vi "prepare_keyboard_notes.vi"(7 "Anticlockwise rotations [0-3] (0)":i32, 8 "error in (no error)":errorcluster, 9 "Note Length (-1)":dbl=-1.0, 10 "Total Length (1200)":dbl=1200.0, 11 "midi-ui in":refnum<class "midi-ui.lvclass">) -> (0 "error out":errorcluster, 3 "midi-ui out":refnum<class "midi-ui.lvclass">)   [LabVIEW 2020, in "midi-ui.lvclass"]
uses:
  midi-ui.lvclass
  midi-ui.lvclass/midi-ui.ctl
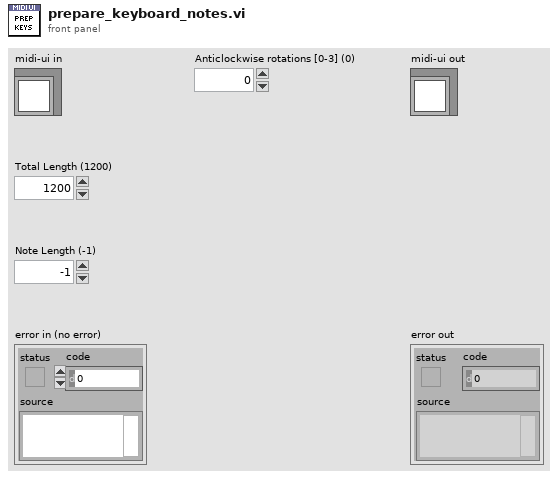
[diagram p1: front panel]
types:
  T1 = typedef "midi-ui.lvclass/privatedata.ctl" = cluster{"White Key Length":dbl, "White Key Width":dbl, "Black Key Length":dbl, "Polygon Corners by Name":map{string, cluster{"x":dbl, "y":dbl}[]}, "Anticlockwise rotations [0-3] (0)":i32, "Polygon Corners by Note Name":map{string, cluster{"x":dbl, "y":dbl}[]}, "Picture Control":refnum<vi>, "Owning VI":refnum<vi>, "Control Index":i32, "Note Bounds by Note Name":map{string, cluster{"max":dbl, "min":dbl}}, "Notes on screen":cluster{"Note Value":enum8{"C-2", "C#-2", "D-2", "D#-2", "E-2", "F-2", "F#-2", "G-2", "G#-2", "A-2", "A#-2", "B-2", "C-1", "C#-1", "D-1", "D#-1", "E-1", "F-1", "F#-1", "G-1", "G#-1", "A-1", "A#-1", "B-1", "C0", "C#0", "D0", "D#0", "E0", "F0", "F#0", "G0", "G#0", "A0", "A#0", "B0", "C1", "C#1", "D1", "D#1", "E1", "F1", "F#1", "G1", "G#1", "A1", "A#1", "B1", "C2", "C#2", "D2", "D#2", "E2", "F2", "F#2", "G2", "G#2", "A2", "A#2", "B2", "C3", "C#3", "D3", "D#3", "E3", "F3", "F#3", "G3", "G#3", "A3", "A#3", "B3", "C4", "C#4", "D4", "D#4", "E4", "F4", "F#4", "G4", "G#4", "A4", "A#4", "B4", "C5", "C#5", "D5", "D#5", "E5", "F5", "F#5", "G5", "G#5", "A5", "A#5", "B5", "C6", "C#6", "D6", "D#6", "E6", "F6", "F#6", "G6", "G#6", "A6", "A#6", "B6", "C7", "C#7", "D7", "D#7", "E7", "F7", "F#7", "G7", "G#7", "A7", "A#7", "B7", "C8", "C#8", "D8", "D#8", "E8", "F8", "F#8", "G"}, "End Time":u32, "Start Time":u32}[], "Polygon Pictures by Note Name":map{i32, cluster{"Note On":picture, "Note Off":picture}}, "keyboard":picture[], "Keyboard Note Index by Name":map{i32, i32}, "music":picture[], "Music Pictures by Index":map{i32, cluster{"Note On":picture, "Note Off":picture}}, "Music Note Index by NoteOnID":map{i32, i32}, "Music Note Index by NoteOffID":map{i32, i32}}
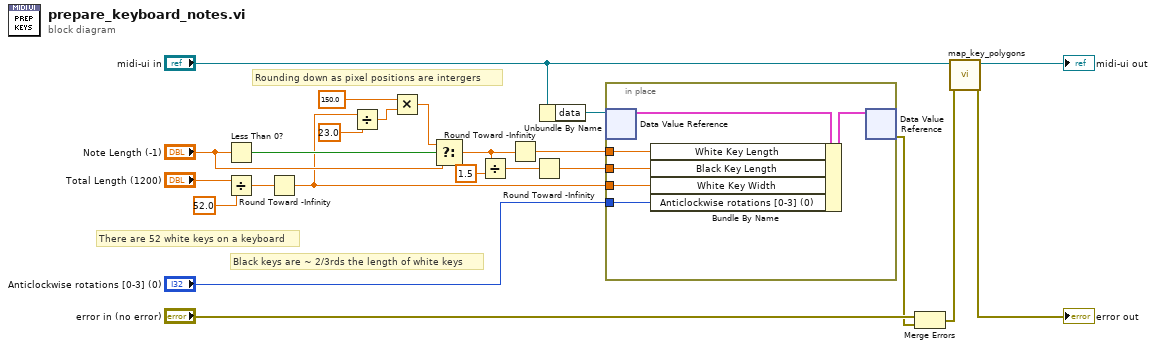
[diagram p0: block diagram]
diagram:
  # "Rounding down as pixel positions are intergers"
  # "Black keys are ~ 2/3rds the length of white keys"
  # "There are 52 white keys on a keyboard"
  n1 = Less Than 0?(x="Note Length (-1)") -> (x < 0?=w18:bool)
  n2 = Divide(x="Total Length (1200)", y=52.0) -> (x/y=w12:dbl)
  n3 = Round Toward -Infinity(1:w12) -> (0:w6:dbl)
  n4 = Divide(x=w6, y=23.0) -> (x/y=w15:dbl)
  n5 = Multiply(x=150.0 ("y"), y=w15) -> (x*y=w13:dbl)
  n6 = Select(t=w13, s=w18, f="Note Length (-1)") -> (s? t:f=w11:dbl)
  n7 = Divide(x=w11, y=1.5) -> (x/y=w10:dbl)
  n8 = Round Toward -Infinity(1:w11) -> (0:w8:dbl)
  n9 = Round Toward -Infinity(1:w10) -> (0:w7:dbl)
  n10 = Unbundle By Name("midi-ui in") -> ("data"=w9:refnum<data-value>)
  n11 = in-place {
    in-place-border: w8 -> [w28]
    in-place-border: w7 -> [w27]
    in-place-border: w6 -> [w26]
    in-place-border: "Anticlockwise rotations [0-3] (0)" -> [w25]
    n12 = in-place-dvr #1(w9) -> (w29:T1)  [unwired: 1 out]
    n13 = Bundle By Name(cluster=w29, "White Key Length"=w28, "Black Key Length"=w27, "White Key Width"=w26, "Anticlockwise rotations [0-3] (0)"=w25) -> (w24:T1)
    n14 = in-place-dvr #1(w24) -> (w2:errorcluster)  [unwired: 1 out]
  }
  n15 = Merge Errors("error in (no error)", w2) -> (w1:errorcluster)
  n16 = call "map_key_polygons.vi"("error in (no error)"=w1, "midi-ui in"="midi-ui in") -> ("error out"=→"error out":errorcluster, "midi-ui out"=→"midi-ui out":refnum<class "midi-ui.lvclass">)  [unwired: 8 in]
